vi "Misssatges finals.vi"(4 "result string in":string, 5 "Boolean":bool, 6 "Numeric 2":u32, 7 "Boolean 2":bool, 8 "error in (no error)":errorcluster, 9 "Numeric":i32, 10 "Boolean 3":bool, 11 "Byte Stream File in":refnum<file>) -> (0 "error out":errorcluster, 2 "result string out":string, 3 "Byte Stream File out":refnum<file>)   [LabVIEW 2023]
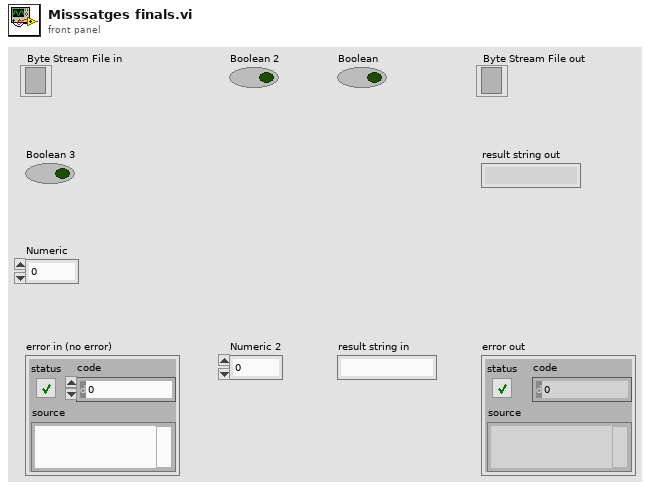
[diagram p1: front panel]
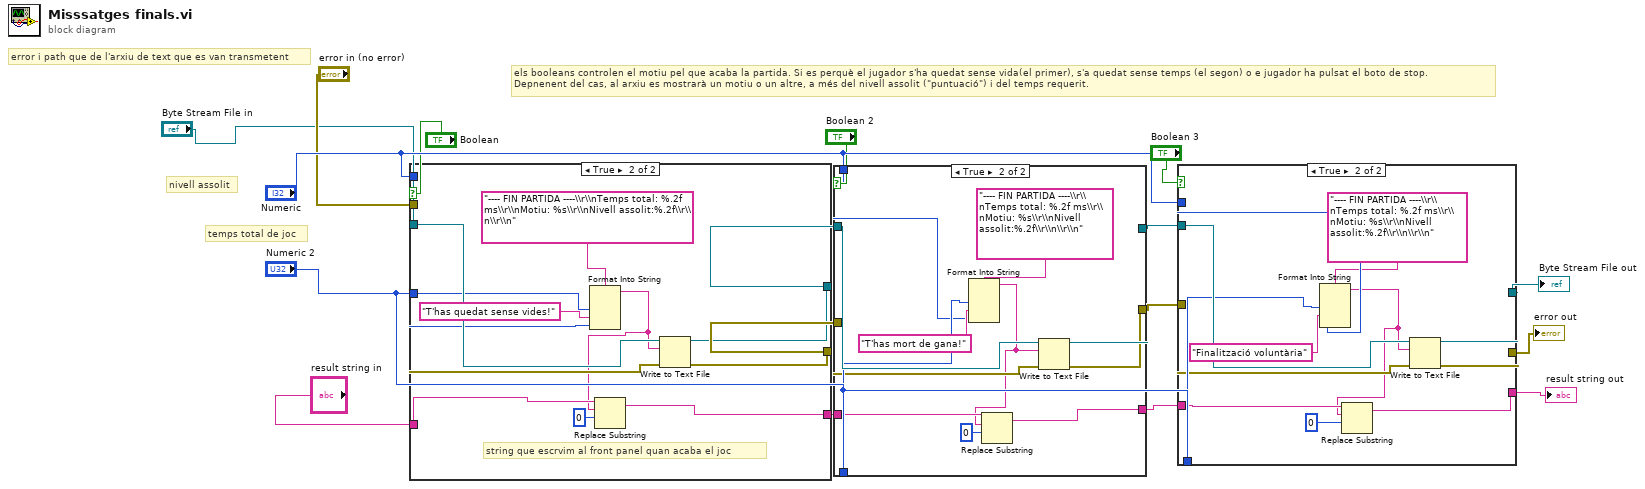
[diagram p0: block diagram]
diagram:
  # "els booleans controlen el motiu pel que acaba la partida. Si es perquè el jugador s'ha quedat sense vida(el primer), s'a quedat sense temps (el segon) o e jugador ha pulsat el boto de stop. \nDepnenent del cas, al arxiu es mostrarà un motiu o un altre, a més del nivell assolit (\"puntuació\") i del temps requerit."
  # "nivell assolit"
  # "temps total de joc"
  # "error i path que de l'arxiu de text que es van transmetent"
  n1 = case shown="True" "Boolean" {
    tunnel: "Byte Stream File in" -> [w20 w31]
    tunnel: "Numeric 2" -> [_ w29]
    tunnel: [w20 w28] -> w7
    tunnel: "error in (no error)" -> [w19 w27]
    tunnel: [w19 w26] -> w10
    tunnel: "Numeric" -> [_ w25]
    tunnel: "result string in" -> [w18 w24]
    tunnel: [w18 w23] -> w14
    frame False {
    }
    frame True {
      # "string que escrvim al front panel quan acaba el joc"
      n2 = Format Into String(format string="---- FIN PARTIDA ----\\r\\nTemps total: %.2f ms\\r\\nMotiu: %s\\r\\nNivell assolit:%.2f\\r\\n\\r\\n", w29, "T'has quedat sense vides!", w25) -> (resulting string=w22:string)  [unwired: 2 in, 1 out]
      n3 = Replace Substring(3:0 ("offset (0)"), 4:w22, 5:w24) -> (1:w23:string)  [unwired: 1 in, 1 out]
      n4 = Write to Text File(file (use dialog)=w31, text=w22, error in=w27) -> (refnum out=w28:refnum<file>, error out=w26:errorcluster)  [unwired: 1 in, 1 out]
    }
  }
  n5 = case shown="True" "Boolean 2" {
    tunnel: w7 -> [w35 w47]
    tunnel: "Numeric 2" -> [_ w45]
    tunnel: [w35 w44] -> w8
    tunnel: w10 -> [w34 w43]
    tunnel: [w34 w42] -> w11
    tunnel: "Numeric" -> [_ w40]
    tunnel: w14 -> [w33 w39]
    tunnel: [w33 w38] -> w15
    frame False {
    }
    frame True {
      n6 = Format Into String(format string="---- FIN PARTIDA ----\\r\\nTemps total: %.2f ms\\r\\nMotiu: %s\\r\\nNivell assolit:%.2f\\r\\n\\r\\n", w45, "T'has mort de gana!", w40) -> (resulting string=w37:string)  [unwired: 2 in, 1 out]
      n7 = Replace Substring(3:0 ("offset (0)"), 4:w37, 5:w39) -> (1:w38:string)  [unwired: 1 in, 1 out]
      n8 = Write to Text File(file (use dialog)=w47, text=w37, error in=w43) -> (refnum out=w44:refnum<file>, error out=w42:errorcluster)  [unwired: 1 in, 1 out]
    }
  }
  n9 = case shown="True" "Boolean 3" {
    tunnel: w8 -> [w50 w62]
    tunnel: "Numeric 2" -> [_ w60]
    tunnel: [w50 w59] -> w1
    tunnel: w11 -> [w49 w58]
    tunnel: [w49 w57] -> w12
    tunnel: "Numeric" -> [_ w56]
    tunnel: w15 -> [w48 w54]
    tunnel: [w48 w53] -> w16
    frame False {
    }
    frame True {
      n10 = Format Into String(format string="---- FIN PARTIDA ----\\r\\nTemps total: %.2f ms\\r\\nMotiu: %s\\r\\nNivell assolit:%.2f\\r\\n\\r\\n", w60, "Finalització voluntària", w56) -> (resulting string=w52:string)  [unwired: 2 in, 1 out]
      n11 = Replace Substring(3:0 ("offset (0)"), 4:w52, 5:w54) -> (1:w53:string)  [unwired: 1 in, 1 out]
      n12 = Write to Text File(file (use dialog)=w62, text=w52, error in=w58) -> (refnum out=w59:refnum<file>, error out=w57:errorcluster)  [unwired: 1 in, 1 out]
    }
  }
  "result string out" <- w16
  "Byte Stream File out" <- w1
  "error out" <- w12
